vi "Test Check Publisher Data Length.vi"() -> ()   [LabVIEW 2021]
uses:
  Iceoryx.lvlib
panel:
  out "pass":bool
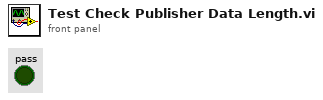
[diagram p1: front panel]
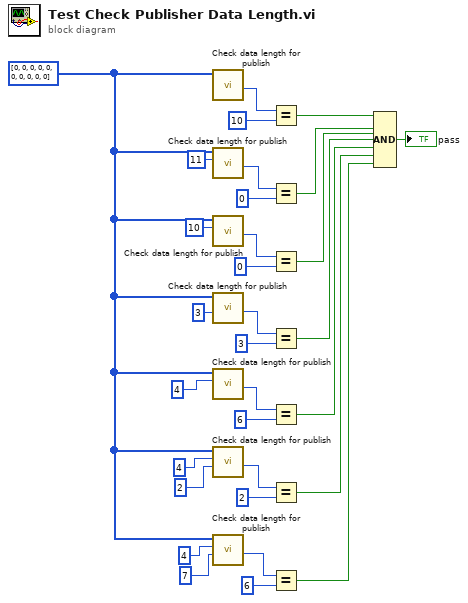
[diagram p0: block diagram]
diagram:
  w9 = u8[] [0, 0, 0, 0, 0, 0, 0, 0, 0, 0] ("Data In")
  n1 = call "Check data length for publish.vi"("Data In"=w9) -> ("Length out"=w31:u32)  [unwired: 8 in, 2 out]
  n2 = call "Check data length for publish.vi"("Offset in"=u32 11, "Data In"=w9) -> ("Length out"=w28:u32)  [unwired: 7 in, 2 out]
  n3 = call "Check data length for publish.vi"("Offset in"=u32 10, "Data In"=w9) -> ("Length out"=w15:u32)  [unwired: 7 in, 2 out]
  n4 = call "Check data length for publish.vi"("Length in"=3, "Data In"=w9) -> ("Length out"=w26:u32)  [unwired: 7 in, 2 out]
  n5 = call "Check data length for publish.vi"("Offset in"=u32 4, "Data In"=w9) -> ("Length out"=w22:u32)  [unwired: 7 in, 2 out]
  n6 = call "Check data length for publish.vi"("Length in"=2, "Offset in"=u32 4, "Data In"=w9) -> ("Length out"=w19:u32)  [unwired: 6 in, 2 out]
  n7 = call "Check data length for publish.vi"("Length in"=7, "Offset in"=u32 4, "Data In"=w9) -> ("Length out"=w11:u32)  [unwired: 6 in, 2 out]
  n8 = Equal?(x=w31, y=u32 10) -> (x = y?=w8:bool)
  n9 = Equal?(x=w28, y=u32 0) -> (x = y?=w7:bool)
  n10 = Equal?(x=w15, y=u32 0) -> (x = y?=w6:bool)
  n11 = Equal?(x=w26, y=u32 3) -> (x = y?=w5:bool)
  n12 = Equal?(x=w22, y=u32 6) -> (x = y?=w4:bool)
  n13 = Equal?(x=w19, y=u32 2) -> (x = y?=w3:bool)
  n14 = Equal?(x=w11, y=u32 6) -> (x = y?=w2:bool)
  n15 = Compound Arithmetic op=AND(w8, w7, w6, w5, w4, w3, w2) -> (→"pass":bool)
